vi "Create Full pubsub Topic Name.vi"(8 "error in":errorcluster, 10 "Topic":string, 11 "Plugin name":string) -> (0 "error out":errorcluster, 3 "Full Topic":string)   [LabVIEW 2021, in "Iceoryx Channel Utilities.lvlib"]
uses:
  Iceoryx Channel Utilities.lvlib
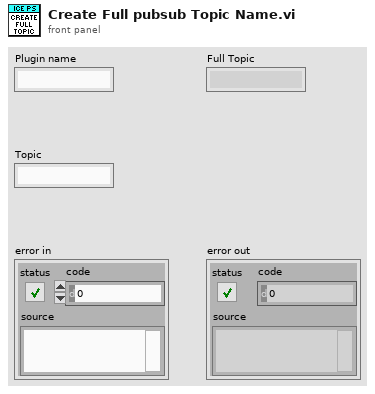
[diagram p1: front panel]
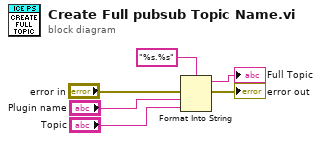
[diagram p0: block diagram]
diagram:
  n1 = Format Into String(format string="%s.%s", error in="error in", "Plugin name", "Topic") -> (resulting string=→"Full Topic":string, error out=→"error out":errorcluster)  [unwired: 1 in]
